vi "Base64_Encode.vi"(10 "error in (no error)":errorcluster, 11 "String":string) -> (2 "error out":errorcluster, 3 "Encoded String":string)   [LabVIEW 2013, in "Serializer.Base64.lvclass"]
uses:
  Serializer.Base64.lvclass
  Serializer.Base64.lvclass/Serializer.Base64.ctl
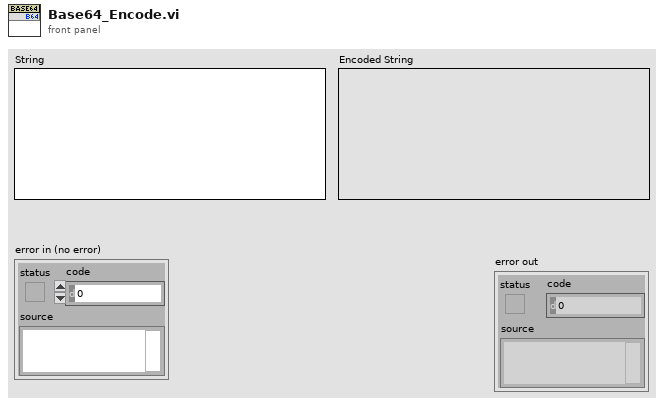
[diagram p1: front panel]
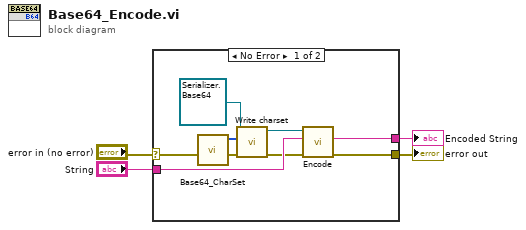
[diagram p0: block diagram]
diagram:
  n1 = case shown="No Error" "error in (no error)" {
    selector: "error in (no error)" -> [w7 w13]
    tunnel: "String" -> [w10 _]
    tunnel: [w9 _] -> w2
    tunnel: [w8 w13] -> w1
    frame No Error {
      n2 = call "Base64_CharSet.vi"() -> ("base64 set"=w12:u8[])  [unwired: 11 in]
      n3 = call "Write charset.vi"("error in (no error)"=w7, "charset"=w12, "Serializer.Base64 in"=refnum<class "Serializer.Base64.lvclass"> refnum) -> ("error out"=w6:errorcluster, "Serializer.Base64 out"=w11:refnum<class "Serializer.Base64.lvclass">)  [unwired: 7 in]
      n4 = call "Encode.vi"("error in (no error)"=w6, "String"=w10, "Serializer.Base64 in"=w11) -> ("error out"=w8:errorcluster, "encoded string"=w9:string)  [unwired: 6 in, 1 out]
    }
    frame Error {
    }
  }
  "Encoded String" <- w2
  "error out" <- w1
